vi "ZM-HWM-stop.vi"(8 "error in (no error)":errorcluster, 11 "ZM-HWM-hardware_manager in":refnum<class "ZM-HWM-hardware_manager.lvclass">) -> (0 "error out":errorcluster, 3 "ZM-HWM-hardware_manager out":refnum<class "ZM-HWM-hardware_manager.lvclass">)   [LabVIEW 2020, in "ZM-HWM-hardware_manager.lvlib" / "ZM-HWM-hardware_manager.lvclass"]
doc: "Stop hook of the hardware manager, called in Actor Core after Call Parent: fires the stop user event, so the loops of ZM-HWM-helperAcquisition end. The error goes on to ZM-HWM-close."
uses:
  ZM-HWM-hardware_manager.lvclass
  ZM-HWM-hardware_manager.lvclass/ZM-HWM-hardware_manager.ctl
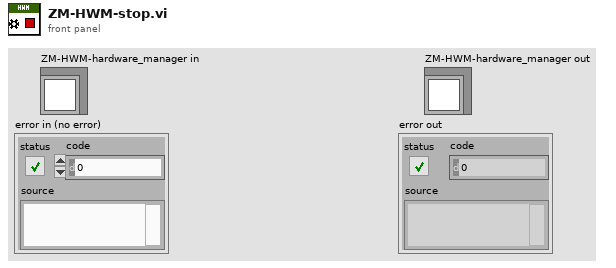
[diagram p1: front panel]
types:
  T1 = typedef "ZM-HWM-hardware_manager.lvlib/ZM-HWM-hardware_manager.lvclass/ZM-HWM-EVENTS.ctl" = cluster{"stop":refnum<user-event>}
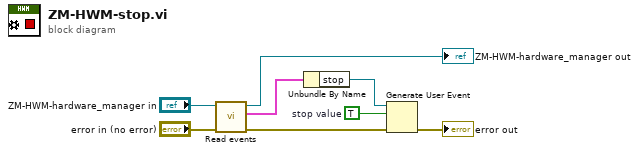
[diagram p0: block diagram]
diagram:
  w4 = TRUE  # stop value
  n1 = call "Read events.vi"("error in (no error)"="error in (no error)", "ZM-HWM-hardware_manager in"="ZM-HWM-hardware_manager in") -> ("error out"=w3:errorcluster, "ZM-HWM-EVENTS"=w6:T1, "ZM-HWM-hardware_manager out"=→"ZM-HWM-hardware_manager out":refnum<class "ZM-HWM-hardware_manager.lvclass">)  [unwired: 7 in]
  n2 = Unbundle By Name(w6) -> ("stop"=w5:refnum<user-event>)
  n3 = Generate User Event(user event=w5, event data cluster=w4, error in=w3) -> (error out=→"error out":errorcluster)  [unwired: 1 in, 1 out]
